vi "LTE Call Handover.vi"(8 "error in (no error)":errorcluster caption="에러 입력(에러 없음)", 10 "LTE Call Handover Param":T1, 11 "Instrument Manager 입력":refnum<class "Instrument Manager.lvclass">) -> (0 "error out":errorcluster caption="에러 출력", 3 "Instrument Manager 출력":refnum<class "Instrument Manager.lvclass">)   [LabVIEW 2023, in "Instrument Manager.lvclass"]
uses:
  Instrument Manager.lvclass
  Type Definition/LTE Call Handover Param.ctl
  Module/ANRITSU Call Box/Type Definition/LTE Supported BandWidth.ctl
  Instrument Manager.lvclass/Instrument Manager.ctl
  4fb08914-a05c-4a83-b6db-b7e92e9bc503.vi
  Module/ANRITSU Call Box/ANRITSU Call Box.lvlib
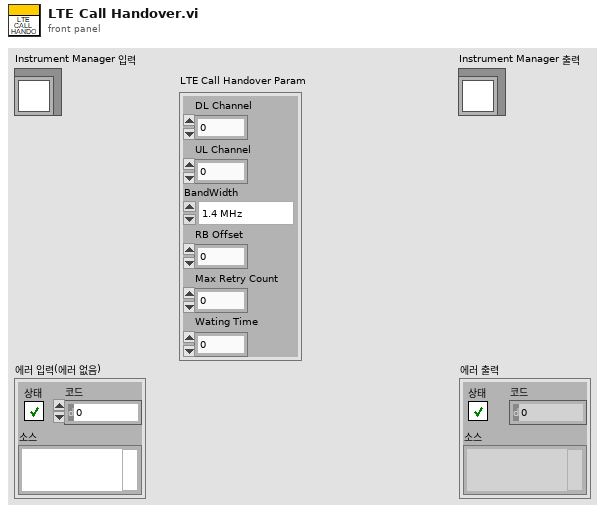
[diagram p1: front panel]
types:
  T1 = typedef "LTE Call Handover Param.ctl" = cluster{"DL Channel":i32, "UL Channel":i32, "BandWidth":T2, "RB Offset":i32, "Max Retry Count":i32, "Wating Time":i32}
  T2 = typedef "ANRITSU Call Box.lvlib/LTE Supported BandWidth.ctl" = enum16{"1.4 MHz", "3 MHz", "5 MHz", "10 MHz", "15 MHz", "20 MHz"}
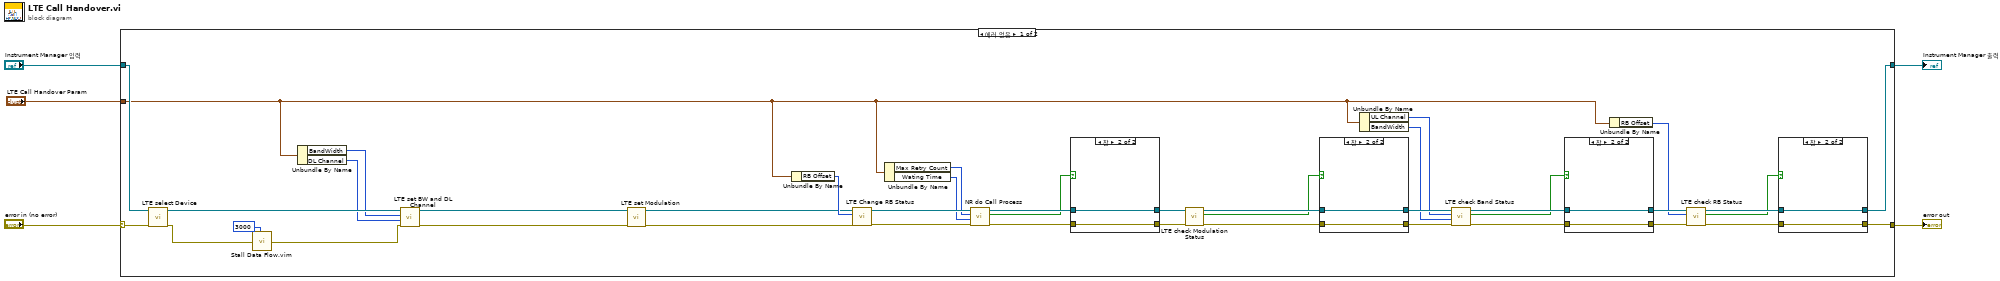
[diagram p0: block diagram]
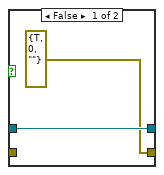
[diagram p2: hidden frame]
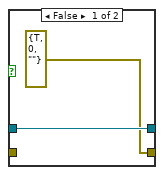
[diagram p3: hidden frame]
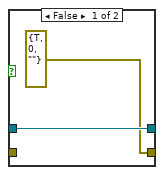
[diagram p4: hidden frame]
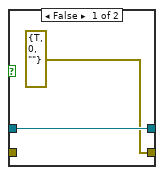
[diagram p5: hidden frame]
diagram:
  n1 = case shown="에러 없음" "error in (no error)" {
    selector: "error in (no error)" -> [w18 w64]
    tunnel: [w20 w64] -> w1
    tunnel: [w19 w63] -> w2
    tunnel: "Instrument Manager 입력" -> [w17 w63]
    tunnel: "LTE Call Handover Param" -> [w14 _]
    frame No Error {
      n2 = call "LTE select Device.vi"("error in (no error)"=w18, "Instrument Manager 입력"=w17) -> ("error out"=w8:errorcluster, "Instrument Manager 출력"=w11:refnum<class "Instrument Manager.lvclass">)  [unwired: 8 in]
      n3 = call "Stall Data Flow.vim"("value in"=w8, "milliseconds to wait"=u32 3000) -> ("value out"=w7:errorcluster)  [unwired: 1 out]
      n4 = Unbundle By Name(w14) -> ("BandWidth"=w9:T2, "DL Channel"=w10:i32)
      n5 = call "LTE set BW and DL Channel.vi"("error in (no error)"=w7, "PCC Downlink"=w10, "BandWidth"=w9, "Instrument Manager 입력"=w11) -> ("error out"=w13:errorcluster, "Instrument Manager 출력"=w12:refnum<class "Instrument Manager.lvclass">)  [unwired: 6 in]
      n6 = call "LTE set Modulation.vi"("error in (no error)"=w13, "Instrument Manager 입력"=w12) -> ("error out"=w16:errorcluster, "Instrument Manager 출력"=w15:refnum<class "Instrument Manager.lvclass">)  [unwired: 8 in]
      n7 = Unbundle By Name(w14) -> ("RB Offset"=w46:i32)
      n8 = call "LTE Change RB Status.vi"("error in (no error)"=w16, "RB Offset"=w46, "Instrument Manager 입력"=w15) -> ("error out"=w45:errorcluster, "Instrument Manager 출력"=w44:refnum<class "Instrument Manager.lvclass">)  [unwired: 7 in]
      n9 = Unbundle By Name(w14) -> ("Max Retry Count"=w42:i32, "Wating Time"=w43:i32)
      n10 = call "NR do Call Process.vi"("error in (no error)"=w45, "Waiting Time"=w43, "Max Retry Count"=w42, "Instrument Manager 입력"=w44) -> ("error out"=w41:errorcluster, "Connected?"=w39:bool, "Instrument Manager 출력"=w40:refnum<class "Instrument Manager.lvclass">)  [unwired: 5 in]
      n11 = case shown="참" w39 {
        tunnel: w40 -> [w60 w62]
        tunnel: [w60 w62] -> w37
        tunnel: [errorcluster {"status"=TRUE, "code"=0, "source"=""} ("error out") w61] -> w38
        tunnel: w41 -> [_ w61]
        frame False {
        }
        frame True {
        }
      }
      n12 = call "LTE check Modulation Status.vi"("error in (no error)"=w38, "Instrument Manager 입력"=w37) -> ("error out"=w36:errorcluster, "불리언"=w34:bool, "Instrument Manager 출력"=w35:refnum<class "Instrument Manager.lvclass">)  [unwired: 7 in]
      n13 = case shown="참" w34 {
        tunnel: w35 -> [w56 w58]
        tunnel: [w56 w58] -> w32
        tunnel: [errorcluster {"status"=TRUE, "code"=0, "source"=""} ("error out") w57] -> w33
        tunnel: w36 -> [_ w57]
        frame False {
        }
        frame True {
        }
      }
      n14 = Unbundle By Name(w14) -> ("UL Channel"=w30:i32, "BandWidth"=w31:T2)
      n15 = call "LTE check Band Status.vi"("error in (no error)"=w33, "BandWidth"=w31, "UL Channel"=w30, "Instrument Manager 입력"=w32) -> ("error out"=w29:errorcluster, "불리언"=w27:bool, "Instrument Manager 출력"=w28:refnum<class "Instrument Manager.lvclass">)  [unwired: 5 in]
      n16 = case shown="참" w27 {
        tunnel: w28 -> [w52 w54]
        tunnel: [w52 w54] -> w25
        tunnel: [errorcluster {"status"=TRUE, "code"=0, "source"=""} ("error out") w53] -> w26
        tunnel: w29 -> [_ w53]
        frame False {
        }
        frame True {
        }
      }
      n17 = Unbundle By Name(w14) -> ("RB Offset"=w24:i32)
      n18 = call "LTE check RB Status.vi"("error in (no error)"=w26, "RB Offset"=w24, "Instrument Manager 입력"=w25) -> ("error out"=w23:errorcluster, "불리언"=w21:bool, "Instrument Manager 출력"=w22:refnum<class "Instrument Manager.lvclass">)  [unwired: 6 in]
      n19 = case shown="참" w21 {
        tunnel: w22 -> [w48 w50]
        tunnel: [w48 w50] -> w19
        tunnel: [errorcluster {"status"=TRUE, "code"=0, "source"=""} ("error out") w49] -> w20
        tunnel: w23 -> [_ w49]
        frame False {
        }
        frame True {
        }
      }
    }
    frame Error {
    }
  }
  "error out" <- w1
  "Instrument Manager 출력" <- w2
